vi "HW XML Tx - Write.vi"(0 "String (in)":string, 1 "Use Octal Labels?":bool, 2 "Selected Channels":i32[](array[numeric]), 3 "Enable Large Schedules?":bool, 5 "formatting (NIVeriStandAdd-Ons)":enum16{"NIVeriStandAdd-Ons", "ni"}(ring), 7 "Parameter Array":T1[](array[typedef])) -> (4 "String (out)":string)   [LabVIEW 2023]
uses:
  Controls/Database_Array.ctl
  Controls/Encoding.ctl
  <userlib>/_OpenG.lib/array/array.llb/Remove Duplicates from 1D Array (I32)__ogtk.vi
  <userlib>/_OpenG.lib/array/array.llb/Filter 1D Array with Scalar (I32)__ogtk.vi
  <userlib>/_OpenG.lib/array/array.llb/Index 1D Array Elements (Variant)__ogtk.vi
  <userlib>/_OpenG.lib/array/array.llb/Remove Duplicates from 1D Array (U32)__ogtk.vi
  <userlib>/_OpenG.lib/array/array.llb/Filter 1D Array with Scalar (U32)__ogtk.vi
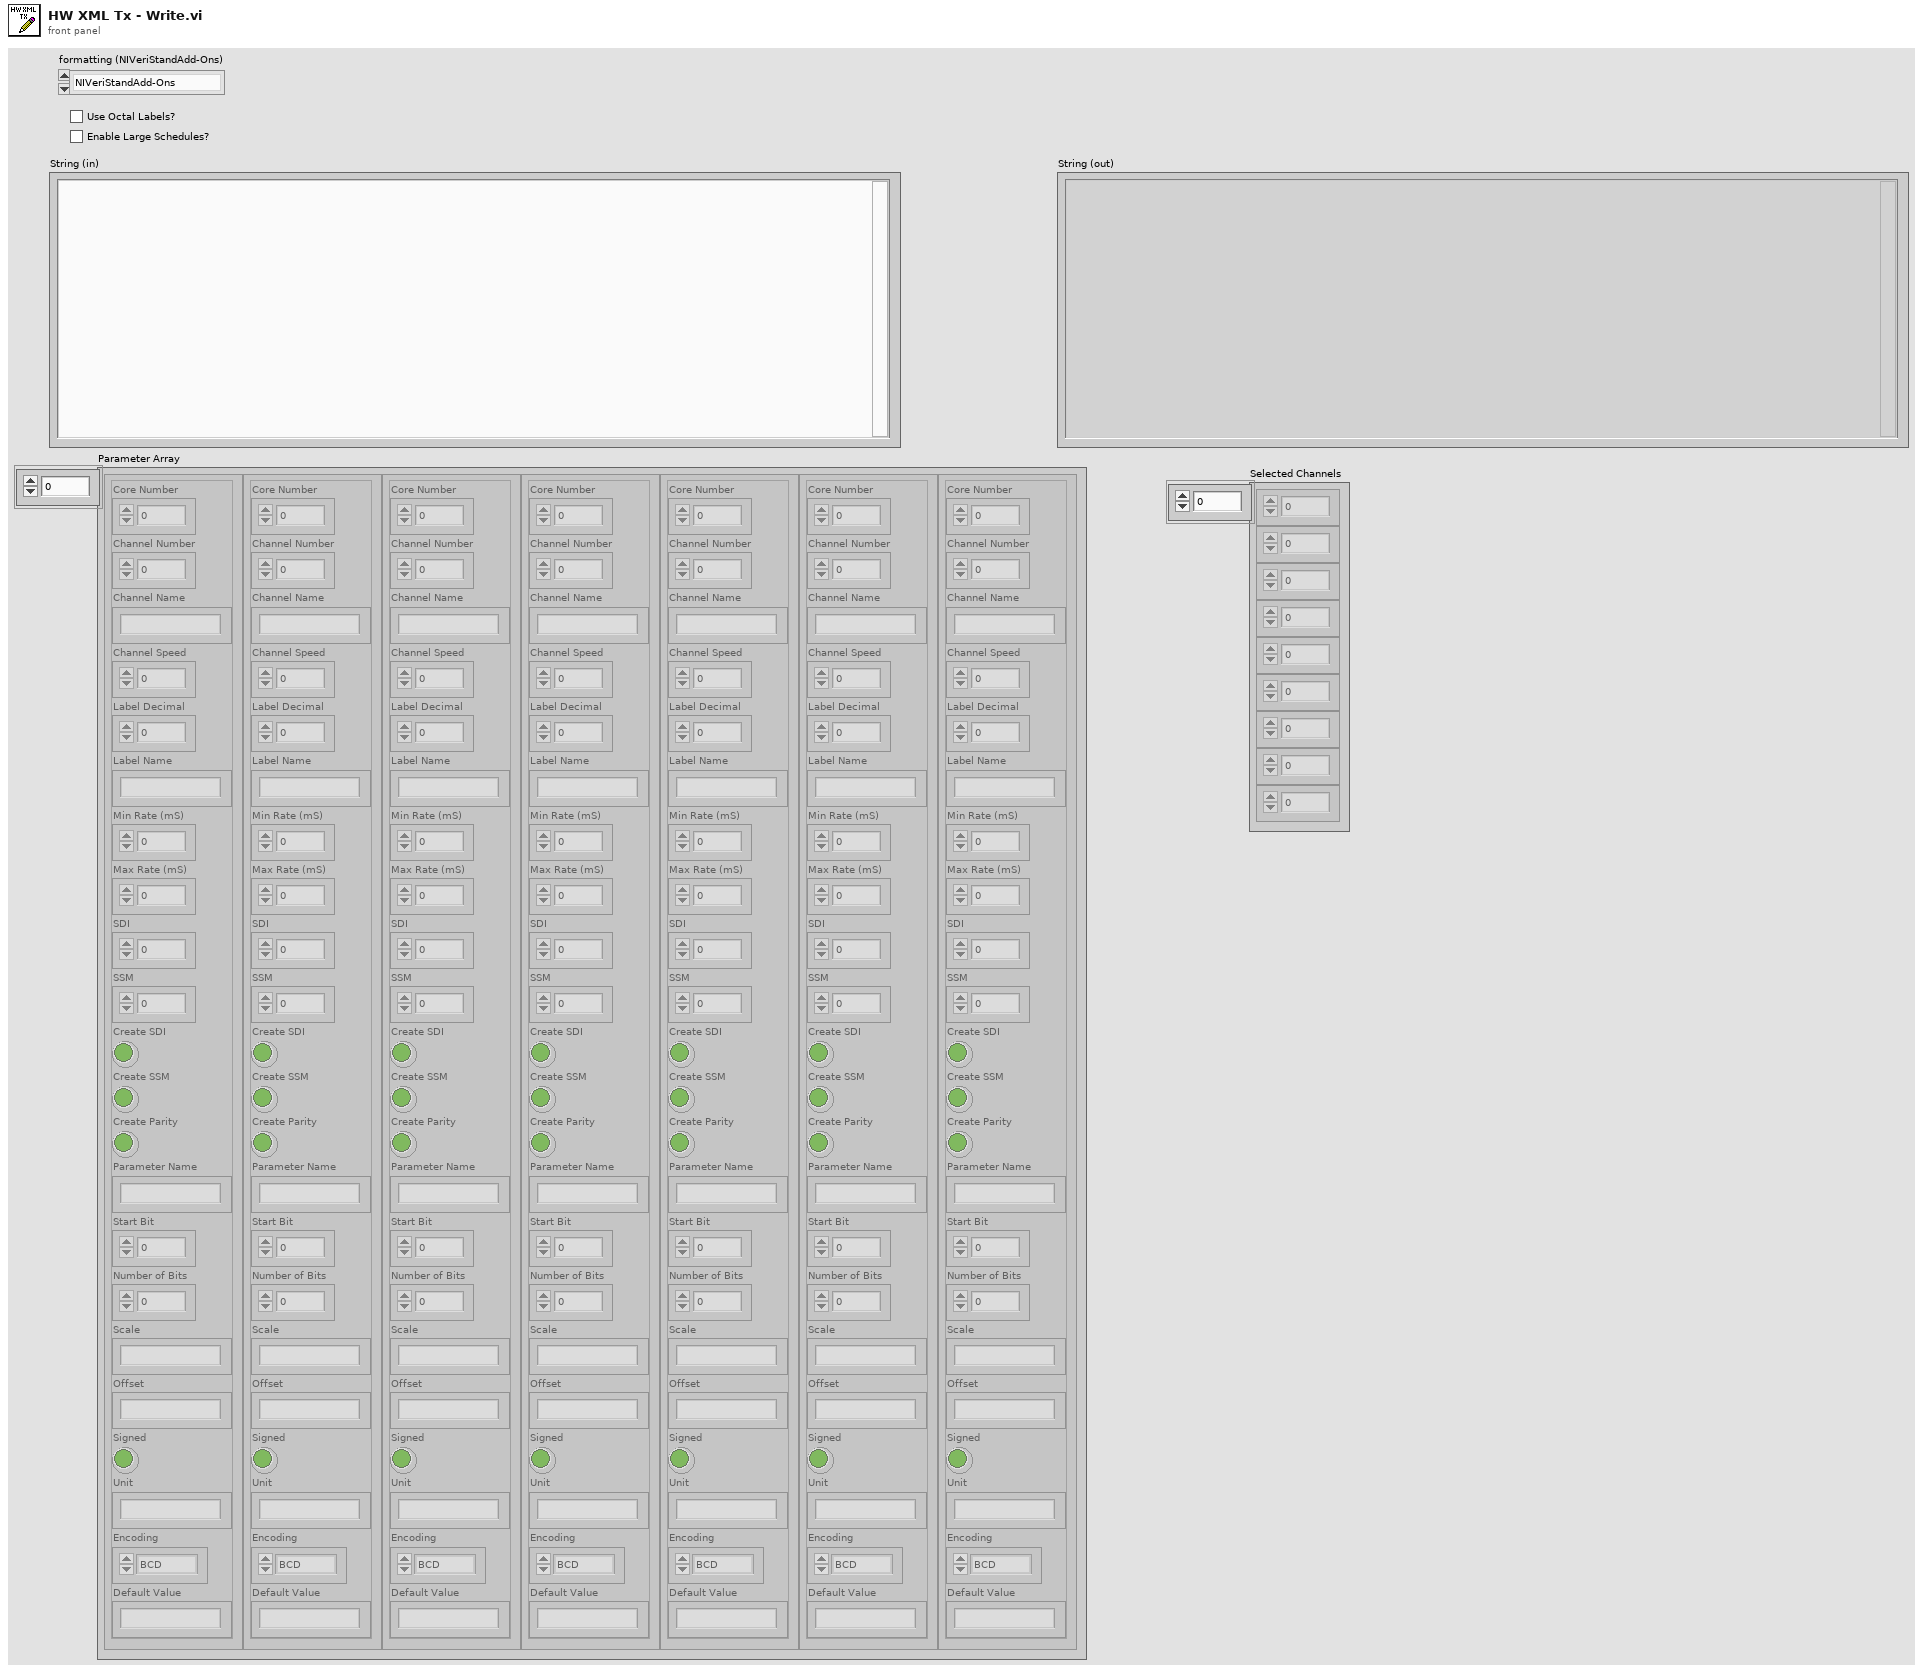
[diagram p1: front panel]
types:
  T1 = typedef "Database_Array.ctl" = cluster{"Core Number":i32, "Channel Number":i32, "Channel Name":string, "Channel Speed":i32, "Label Decimal":u32, "Label Name":string, "Min Rate (mS)":i32, "Max Rate (mS)":i32, "SDI":i32, "SSM":i32, "Create SDI":bool, "Create SSM":bool, "Create Parity":bool, "Parameter Name":string, "Start Bit":i32, "Number of Bits":i32, "Scale":string, "Offset":string, "Signed":bool, "Unit":string, "Encoding":T2, "Default Value":string}
  T2 = typedef "Encoding.ctl" = enum16{"BCD", "BNR", "Discrete"}
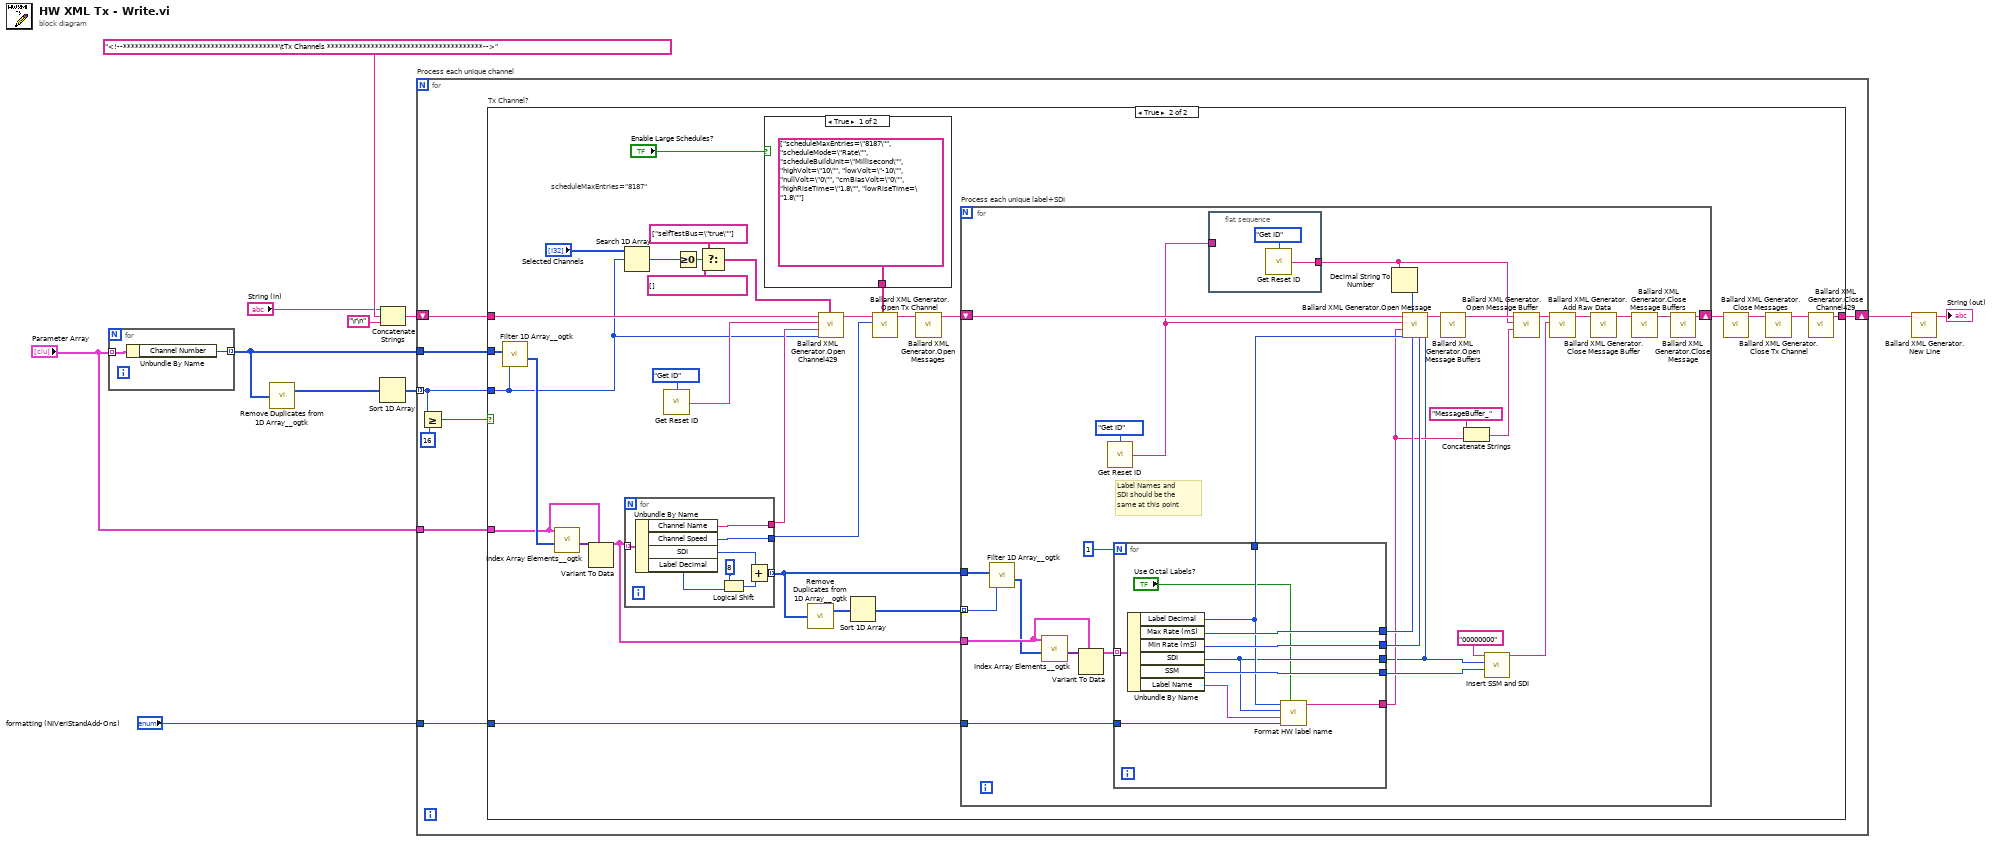
[diagram p0: block diagram]
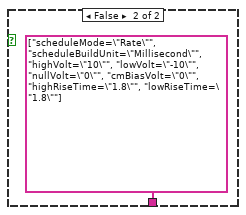
[diagram p3: hidden frame]
diagram:
  n1 = for {
    tunnel: [w13] -> w3 mode=indexing
    tunnel: "Parameter Array" -> [w12] mode=indexing
    n2 = Unbundle By Name(w12) -> ("Channel Number"=w13:i32)
  }
  n3 = call-poly <userlib>:"Remove Duplicates from 1D Array__ogtk.vi"("Input Array"=w3) -> ("Output Array"=w10:i32[])  [unwired: 1 out]
  n4 = Sort 1D Array(array=w10) -> (sorted array=w11:i32[])
  n5 = Concatenate Strings("String (in)", "<!--***************************************\tTx Channels ***************************************-->", "\r\n") -> (w7:string)
  n6 = for "Process each unique channel" {
    tunnel: w11 -> [w18] mode=indexing
    tunnel: w3 -> [w21]
    shift-right: [w19] -> w2
    shift-left: w7 -> [w20]
    tunnel: "Parameter Array" -> [w15]
    tunnel: "formatting (NIVeriStandAdd-Ons)" -> [w14]
    n7 = Greater Or Equal?(x=w18, y=16) -> (x >= y?=w17:bool)
    n8 = case "Tx Channel?" shown="True" w17 {
      tunnel: w21 -> [_ w52]
      tunnel: w20 -> [w22 w49]
      tunnel: [w22 w42] -> w19
      tunnel: w18 -> [_ w26]
      tunnel: w15 -> [_ w36]
      tunnel: w14 -> [_ w24]
      frame False {
      }
      frame True {
        # "scheduleMaxEntries=\"8187\""
        n9 = call-poly <userlib>:"Filter 1D Array__ogtk.vi"("items to filter"=w26, "array"=w52) -> ("filtered item indices"=w40:i32[])  [unwired: 4 in, 1 out]
        n10 = call-poly <userlib>:"Index Array Elements__ogtk.vi"("indices"=w40, "array"=w36) -> ("elements"=w39:variant[])  [unwired: 9 in]
        n11 = Variant To Data(type=w36, Variant=w39) -> (data=w35:T1[])  [unwired: 1 in, 1 out]
        n12 = Search 1D Array(1D array="Selected Channels", element=w26) -> (index of element=w30:i32)  [unwired: 1 in]
        n13 = for {
          tunnel: w35 -> [w62] mode=indexing
          tunnel: [w61] -> w38
          tunnel: [w60] -> w37
          tunnel: [w55] -> w34 mode=indexing
          n14 = Unbundle By Name(w62) -> ("Channel Name"=w61:string, "Channel Speed"=w60:i32, "SDI"=w57:i32, "Label Decimal"=w56:u32)
          n15 = Logical Shift(y=i16 8, x=w56) -> (x << y=w59:u32)
          n16 = Add(x=w57, y=w59) -> (x+y=w55:u32)
        }
        n17 = call "Get Reset ID.vi"("Function"=enum16{"Get ID", "Reset ID"}."Get ID") -> ("ID"=w33:string)  [unwired: 14 in]
        n18 = Greater Or Equal To 0?(x=w30) -> (x >= 0?=w31:bool)
        n19 = Select(t=string[] ["selfTestBus=\"true\""] ("other params"), s=w31, f=string[] [] ("other params")) -> (s? t:f=w25:string[])
        n20 = case shown="True" "Enable Large Schedules?" {
          tunnel: [string[] ["scheduleMaxEntries=\"8187\"", "scheduleMode=\"Rate\"", "scheduleBuildUnit=\"Millisecond\"", "highVolt=\"10\"", "lowVolt=\"-10\"", "nullVolt=\"0\"", "cmBiasVolt=\"0\"", "highRiseTime=\"1.8\"", "lowRiseTime=\"1.8\""] ("other params") string[] ["scheduleMode=\"Rate\"", "scheduleBuildUnit=\"Millisecond\"", "highVolt=\"10\"", "lowVolt=\"-10\"", "nullVolt=\"0\"", "cmBiasVolt=\"0\"", "highRiseTime=\"1.8\"", "lowRiseTime=\"1.8\""] ("other params")] -> w41
          frame True {
          }
          frame False {
          }
        }
        n21 = call-poly <userlib>:"Remove Duplicates from 1D Array__ogtk.vi"("Input Array"=w34) -> ("Output Array"=w51:u32[])  [unwired: 1 out]
        n22 = call "Ballard XML Generator.Open Channel429.vi"("other params"=w25, "hardware channel"=w26, "name"=w38, "id"=w33, "string in"=w49) -> ("string out"=w47:string)  [unwired: 6 in]
        n23 = Sort 1D Array(array=w51) -> (sorted array=w50:u32[])
        n24 = call "Ballard XML Generator.Open Tx Channel.vi"("other params"=w41, "speedKHz"=w37, "string in"=w47) -> ("string out"=w48:string)  [unwired: 8 in]
        n25 = call "Ballard XML Generator.Open Messages.vi"("string in"=w48) -> ("string out"=w46:string)  [unwired: 10 in]
        n26 = for "Process each unique label+SDI" {
          tunnel: w50 -> [w90] mode=indexing
          tunnel: w34 -> [w92]
          shift-right: [w81] -> w45
          shift-left: w46 -> [w91]
          tunnel: w35 -> [w74]
          tunnel: w24 -> [w63]
          # "Label Names and SDI should be the same at this point"
          n27 = call-poly <userlib>:"Filter 1D Array__ogtk.vi"("items to filter"=w90, "array"=w92) -> ("filtered item indices"=w73:i32[])  [unwired: 4 in, 1 out]
          n28 = call-poly <userlib>:"Index Array Elements__ogtk.vi"("indices"=w73, "array"=w74) -> ("elements"=w77:variant[])  [unwired: 9 in]
          n29 = Variant To Data(type=w74, Variant=w77) -> (data=w76:T1[])  [unwired: 1 in, 1 out]
          n30 = call "Get Reset ID.vi"("Function"=enum16{"Get ID", "Reset ID"}."Get ID") -> ("ID"=w64:string)  [unwired: 14 in]
          n31 = for {
            N: 1 -> [_]
            tunnel: w76 -> [w104] mode=indexing
            tunnel: [w103] -> w72
            tunnel: [w102] -> w71
            tunnel: [w99] -> w67
            tunnel: [w101] -> w70
            tunnel: [w100] -> w69
            tunnel: [w97] -> w68
            tunnel: w63 -> [w96]
            n32 = Unbundle By Name(w104) -> ("Label Decimal"=w100:u32, "Max Rate (mS)"=w103:i32, "Min Rate (mS)"=w102:i32, "SDI"=w99:i32, "SSM"=w101:i32, "Label Name"=w98:string)
            n33 = call "Format HW label name.vi"("Use Octal Channel Names?"="Use Octal Labels?", "formatting"=w96, "Label Name in"=w98, "SDI"=w99, "Label Decimal"=w100) -> ("Label Name out"=w97:string)  [unwired: 6 in]
          }
          n34 = flat-sequence {
            tunnel: [w94] -> w65
            tunnel: w64 -> [_]
            frame #0 {
              n35 = call "Get Reset ID.vi"("Function"=enum16{"Get ID", "Reset ID"}."Get ID") -> ("ID"=w94:string)  [unwired: 14 in]
            }
          }
          n36 = Decimal String To Number(string=w65) -> (number=w80:i32)  [unwired: 2 in, 1 out]
          n37 = call "Ballard XML Generator.Open Message.vi"("SDI"=w67, "minRate (400)"=w71, "maxRate (400)"=w72, "messageBufferIDRef (128)"=w80, "labelDecimal"=w69, "name"=w68, "id"=w64, "string in"=w91) -> ("string out"=w89:string)  [unwired: 3 in]
          n38 = call "Ballard XML Generator.Open Message Buffers.vi"("string in"=w89) -> ("string out"=w88:string)  [unwired: 10 in]
          n39 = Concatenate Strings("MessageBuffer_" ("name"), w68) -> (w86:string)
          n40 = call "Insert SSM and SDI.vi"("SSM"=w70, "SDI"=w67, "Hex (in)"="00000000" ("raw data")) -> ("Hex (out)"=w78:string)  [unwired: 8 in]
          n41 = call "Ballard XML Generator.Open Message Buffer.vi"("name"=w86, "id"=w65, "string in"=w88) -> ("string out"=w82:string)  [unwired: 8 in]
          n42 = call "Ballard XML Generator.Add Raw Data.vi"("raw data"=w78, "string in"=w82) -> ("string out"=w83:string)  [unwired: 9 in]
          n43 = call "Ballard XML Generator.Close Message Buffer.vi"("string in"=w83) -> ("string out"=w84:string)  [unwired: 10 in]
          n44 = call "Ballard XML Generator.Close Message Buffers.vi"("string in"=w84) -> ("string out"=w85:string)  [unwired: 10 in]
          n45 = call "Ballard XML Generator.Close Message.vi"("string in"=w85) -> ("string out"=w81:string)  [unwired: 10 in]
        }
        n46 = call "Ballard XML Generator.Close Messages.vi"("string in"=w45) -> ("string out"=w44:string)  [unwired: 10 in]
        n47 = call "Ballard XML Generator.Close Tx Channel.vi"("string in"=w44) -> ("string out"=w43:string)  [unwired: 10 in]
        n48 = call "Ballard XML Generator.Close Channel429.vi"("string in"=w43) -> ("string out"=w42:string)  [unwired: 10 in]
      }
    }
  }
  n49 = call "Ballard XML Generator.New Line.vi"("string in"=w2) -> ("string out"=→"String (out)":string)  [unwired: 10 in]
